vi "GetApiKeys.vi"(8 "error in (no error)":errorcluster, 11 "ITool in":refnum<class "ITool.lvclass">) -> (0 "error out":errorcluster, 2 "ApiKeys":string[](array[string]), 3 "ITool out":refnum<class "ITool.lvclass">)   [LabVIEW 2017, in "ITool.lvclass"]
uses:
  ITool.lvclass
  ITool.lvclass/ITool.ctl
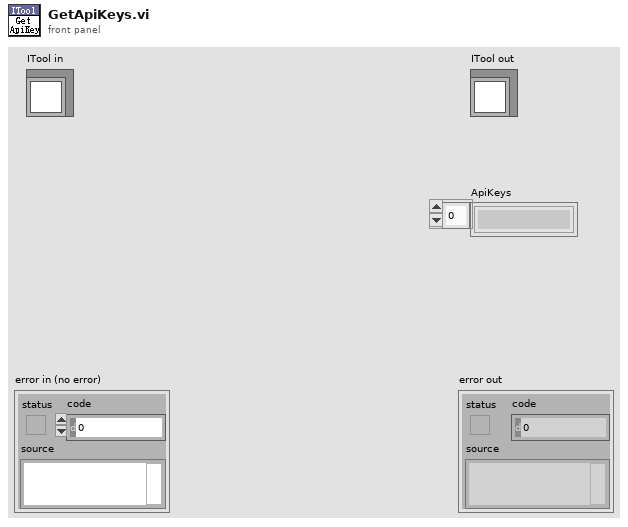
[diagram p1: front panel]
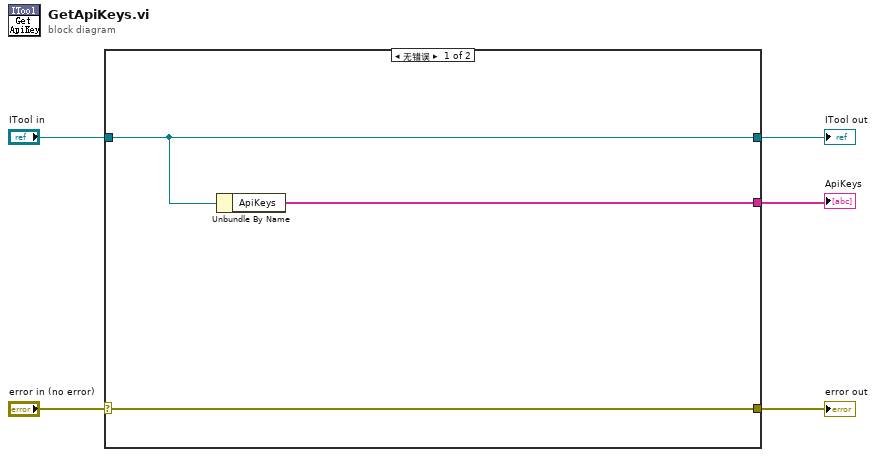
[diagram p0: block diagram]
diagram:
  n1 = case shown="无错误" "error in (no error)" {
    selector: "error in (no error)" -> [w8 w10]
    tunnel: [w8 w10] -> w3
    tunnel: [w7 w9] -> w4
    tunnel: "ITool in" -> [w7 w9]
    tunnel: [w6 _] -> w1
    frame No Error {
      n2 = Unbundle By Name(w7) -> ("ApiKeys"=w6:string[])
    }
    frame Error {
    }
  }
  "ITool out" <- w4
  "error out" <- w3
  "ApiKeys" <- w1
